vi "[ex ce] Show XY graphs.vi"() -> ()   [LabVIEW 2021]
doc: "<B>Example for CalcExpress script syntax</B>\n\nThis simplest example computes some curves and displays them in a probe window with XY Graph. It uses <B>polymorphism</B> of CalcExpress operators and functions to perform computation.\n\n::: CalcExpress Toolkit :::\nCopyright (c) 2000-2026 Konstantin Shifershteyn. All rights reserved."
panel:
  in  "Expression":string="XYGraph();                     //clear graph\n\n// to draw a circle\ni = nvecifn(0, pi(2), 1000);   //values from 0 to pi*2\nk = 9;\nX = k * sin(i);\nY = k * cos(i);\nXYGraph(0, X,Y);               //display plot\n\n// to draw a spiral\ni = nvecifn(0, pi(10), 1000);  //values from 0 to pi*10\nj = i/4;\nX = j * sin(i);\nY = j * cos(i);\nXYGraph(1, X,Y);               //display plot\n\n// to draw a hypocycloid\na=1, b=5, k=2;\ni = nvecifn(0, pi(2), 1000);   //values from 0 to pi*2\nX = (a+b)*cos(i) + k*a*cos((a+b)*i/a);\nY = (a+b)*sin(i) - k*a*sin((a+b)*i/a);\nXYGraph(4, X,Y );             //display plot\n"
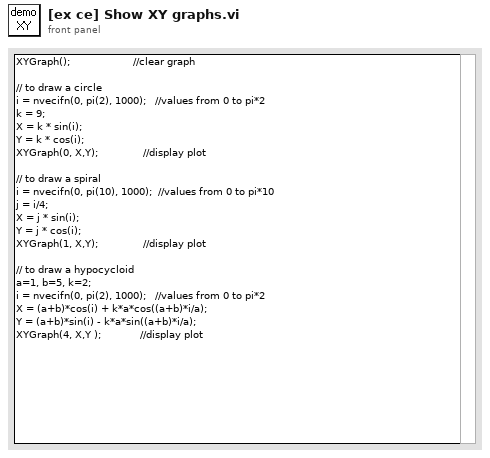
[diagram p1: front panel]
types:
  T1 = typedef "VarMan Variable Context Handle.ctl" = i32
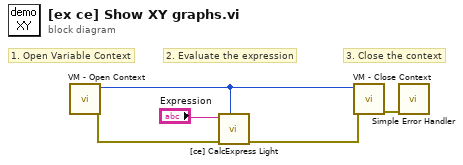
[diagram p0: block diagram]
diagram:
  # "3. Close the context"
  # "2. Evaluate the expression"
  # "1. Open Variable Context"
  n1 = call "VM - Open Context.vi"() -> ("error out"=w4:errorcluster, "VC Handle out"=w1:T1)  [unwired: 9 in, 1 out]
  n2 = call "[ce] CalcExpress Light.vi"("VC Handle"=w1, "error in"=w4, "expression"="Expression") -> ("error out"=w3:errorcluster)  [unwired: 6 in, 2 out]
  n3 = call "VM - Close Context.vi"("error in"=w3, "VC Handle"=w1) -> ("error out"=w2:errorcluster)  [unwired: 8 in, 1 out]
  n4 = call <vilib>:"Simple Error Handler.vi"("error in (no error)"=w2) -> ()  [unwired: 4 in, 5 out]
